vi "Launch Fixture.vi"(11 "Command line args":string[](array[string])) -> (2 "Output":string, 3 "Return code":i32)   [LabVIEW 2020]
doc: "Starts tests\\fixtures\\RemoteVI Fixture.vi (next to this VI) with its values reset to default (a fixture still in memory would keep the last run's) and its front panel open, without waiting for it, then asks RemoteVI Status.vi every 500 ms until the fixture shares port 8089 and returns that share's link with its access token in Output (Return code 0); after 60 s Return code is 1. Its connector pane is the one NI's LabVIEW CLI expects from RunVI (pattern 4815, Command line args at 11, Output at 2, Return code at 3), so tools\\run-lv-integration.ps1 starts the fixture with LabVIEWCLI -OperationName RunVI and reads the link from its output - no ActiveX."
uses:
  source/RemoteVI.lvlib
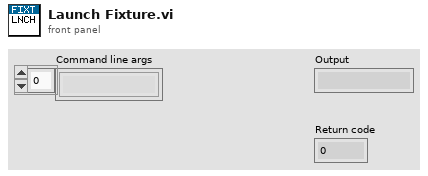
[diagram p1: front panel]
types:
  T1 = cluster{"port":u16, "url":string, "target":string, "kind":string, "whole network":bool, "running":bool, "uptime s":dbl, "clients":cluster{"address":string, "connected s":dbl, "idle s":dbl}[], "fps":dbl, "kB per s":dbl, "frames":u32, "latency ms":dbl, "view only":bool, "last error":string, "hWnd":u64}[]
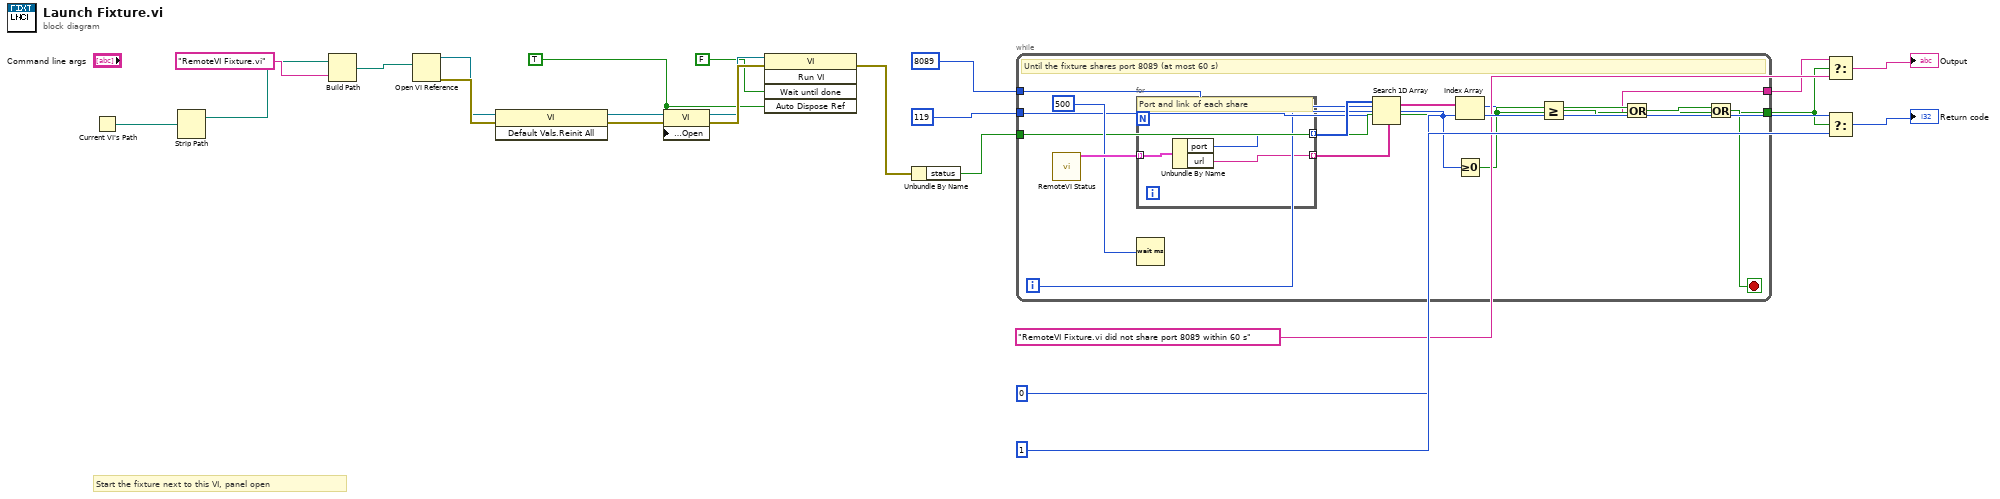
[diagram p0: block diagram]
diagram:
  w7 = TRUE
  # "Start the fixture next to this VI, panel open"
  n1 = Current VI's Path() -> (path=w1:path)
  n2 = Strip Path(path=w1) -> (stripped path=w2:path)  [unwired: 1 out]
  n3 = Build Path(base path=w2, name or relative path="RemoteVI Fixture.vi") -> (appended path=w4:path)
  n4 = Open VI Reference(vi path=w4) -> (vi reference=w5:refnum<vi>, error out=w6:errorcluster)  [unwired: 5 in]
  n5 = invoke class="VI" method="Default Vals.Reinit All"(reference=w5, error in=w6) -> (reference out=w9:refnum<vi>, error out=w10:errorcluster)  [unwired: 1 in, 1 out]
  n6 = property class="VI"(reference=w9, error in=w10, "Front Panel Window:Open"=w7) -> (reference out=w11:refnum<vi>, error out=w12:errorcluster)
  n7 = invoke class="VI" method="Run VI"(reference=w11, error in=w12, "Wait until done"=FALSE, "Auto Dispose Ref"=w7) -> (error out=w13:errorcluster)  [unwired: 1 in, 4 out]
  n8 = Unbundle By Name(w13) -> ("status"=w14:bool)
  n9 = while {
    tunnel: u16 8089 -> [w25]
    tunnel: 119 -> [w26]
    tunnel: [w33] -> w17
    tunnel: [w34] -> w18
    tunnel: w14 -> [w27]
    i -> [w24]
    stop <- w37 stop-if-true
    # "Until the fixture shares port 8089 (at most 60 s)"
    n10 = call "RemoteVI Status.vi"() -> ("servers"=w29:T1)  [unwired: 14 in, 1 out]
    n11 = for {
      tunnel: w29 -> [w38] mode=indexing
      tunnel: [w39] -> w30 mode=indexing
      tunnel: [w40] -> w31 mode=indexing
      # "Port and link of each share"
      n12 = Unbundle By Name(w38) -> ("port"=w39:u16, "url"=w40:string)
    }
    n13 = Wait (ms)(milliseconds to wait=u32 500) -> ()  [unwired: 1 out]
    n14 = Search 1D Array(1D array=w30, element=w25) -> (index of element=w32:i32)  [unwired: 1 in]
    n15 = Index Array(array=w31, index=w32) -> (element=w33:string)
    n16 = Greater Or Equal To 0?(x=w32) -> (x >= 0?=w34:bool)
    n17 = Greater Or Equal?(x=w24, y=w26) -> (x >= y?=w35:bool)
    n18 = Or(x=w34, y=w35) -> (x .or. y?=w36:bool)
    n19 = Or(x=w36, y=w27) -> (x .or. y?=w37:bool)
  }
  n20 = Select(t=w17, s=w18, f="RemoteVI Fixture.vi did not share port 8089 within 60 s") -> (s? t:f=→"Output":string)
  n21 = Select(t=0, s=w18, f=1) -> (s? t:f=→"Return code":i32)
